vi "Read Builder Reference.vi"(8 "error in (no error)":errorcluster, 11 "ToastBuilder in":refnum<class "ToastBuilder.lvclass">) -> (0 "error out":errorcluster, 2 "new reference":T1, 3 "ToastBuilder out":refnum<class "ToastBuilder.lvclass">)   [LabVIEW 2026, in "ToastNotification.lvlib" / "ToastBuilder.lvclass"]
doc: "Private native data-member read accessor for Builder Reference. Return a borrowed alias of the stored .NET handle and pass the class and error through. Does not clone, allocate or close the builder. Use through the class property node in business methods."
uses:
  ToastBuilder.lvclass
  Builder Reference.ctl
  C:/Users/loicw/Documents/LabVIEW/ToastNotifications/Sources/bins/Microsoft.Toolkit.Uwp.Notifications.dll
  bins/Microsoft.Toolkit.Uwp.Notifications.dll
  ToastBuilder.lvclass/ToastBuilder.ctl
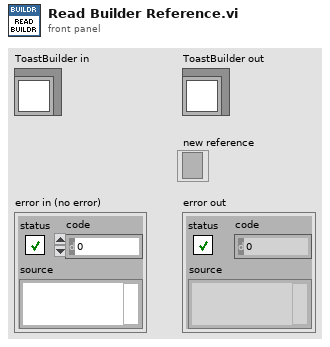
[diagram p1: front panel]
types:
  T1 = typedef "ToastNotification.lvlib/ToastBuilder.lvclass/Builder Reference.ctl" = refnum<k24>
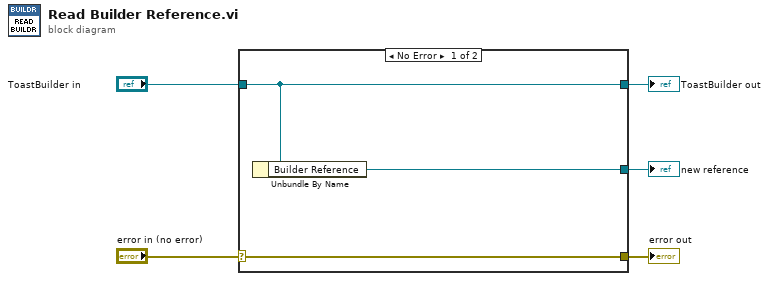
[diagram p0: block diagram]
diagram:
  n1 = case shown="No Error" "error in (no error)" {
    selector: "error in (no error)" -> [w8 w9]
    tunnel: [w8 w9] -> w4
    tunnel: [w7 w10] -> w2
    tunnel: "ToastBuilder in" -> [w7 w10]
    tunnel: [w6 _] -> w1
    frame No Error {
      n2 = Unbundle By Name(w7) -> ("Builder Reference"=w6:T1)
    }
    frame Error {
    }
  }
  "error out" <- w4
  "ToastBuilder out" <- w2
  "new reference" <- w1
